vi "PathPlanner_Path_FromJSON.vi"(11 "JSON String":string) -> (0 "Error":bool, 2 "version":string, 3 "PathPlannerPath":T1={"Reversed"=FALSE, "RotationTargets"=[], "ConstraintZones"=[], "EventMarkers"=[], "GlobalConstraints"={"MaxVelocityMps;"=0.0, "MaxAccelerationMpsSq;"=0.0, "MaxAngularVelRadPsEc;"=0.0, "MaxAngularAccRadPSecSq"=0.0, "Exists"=FALSE, "Unlimited"=FALSE, "NominalVoltageVolts"=12.0}, "GoalEndState"={"VelocityMPS"=0.0, "Rotation"={"VALUE"=0.0, "COS"=1.0, "SIN"=0.0}}, "AllPoints"=[], "Name"="", "Waypoints"=[], "PointTowardsZones"=[], "IdealStartingState"={"VelocityMPS"=0.0, "Rotation"={"VALUE"=1.0, "COS"=0.0, "SIN"=0.0}}, "IsChoreoPath"=FALSE, "PreventFlipping"=FALSE} {"IdealStartingState"."Rotation"."SIN" format="%13.4f"; "IdealStartingState"."Rotation"."COS" format="%13.4f"; "IdealStartingState"."Rotation"."VALUE" format="%13.4f"; "PointTowardsZones"."TargetPosition"."Y" format="%14.3f"; "PointTowardsZones"."TargetPosition"."X" format="%14.3f"; "PointTowardsZones"."RotationOffset"."SIN" format="%13.4f"; "PointTowardsZones"."RotationOffset"."COS" format="%13.4f"; "PointTowardsZones"."RotationOffset"."VALUE" format="%13.4f"; "Waypoints"."nextControl"."Y" format="%14.3f"; "Waypoints"."nextControl"."X" format="%14.3f"; "Waypoints"."anchor"."Y" format="%14.3f"; "Waypoints"."anchor"."X" format="%14.3f"; "Waypoints"."prevControl"."Y" format="%14.3f"; "Waypoints"."prevControl"."X" format="%14.3f"; "AllPoints"."RotationTarget"."rotation"."SIN" format="%13.4f"; "AllPoints"."RotationTarget"."rotation"."COS" format="%13.4f"; "AllPoints"."RotationTarget"."rotation"."VALUE" format="%13.4f"; "AllPoints"."Position"."Y" format="%14.3f"; "AllPoints"."Position"."X" format="%14.3f"; "GoalEndState"."Rotation"."SIN" format="%13.4f"; "GoalEndState"."Rotation"."COS" format="%13.4f"; "GoalEndState"."Rotation"."VALUE" format="%13.4f"; "RotationTargets"."rotation"."SIN" format="%13.4f"; "RotationTargets"."rotation"."COS" format="%13.4f"; "RotationTargets"."rotation"."VALUE" format="%13.4f"})   [LabVIEW 2019, in "PathPlanner24.lvlib"]
doc: "Load a path from a JSON string.\n\nInputs: \n - JSON String - string- The string containing the path definition.\n\nOutputs:\n - Path - cluster - PathPlannerPath created from the given JSON string\n - version - string - version string from JSON\n - Error out - cluster - Error cluster\n\n\nNotes:\n--------\nCurrently the only type of commands that can be issued are Boolean commands. The value is forced to TRUE when the command is issued.\n\nThe following table lists the actions performed for different types of commands:\n - Unknown - nothing - not supported.\n - Wait - nothing - not supported\n - Named - Issue boolean command with TRUE value using the \"name\" as the command name.\n - Path - nothing - not supported\n - Sequential, Parallel, Race, Deadline - Issue boolean command with TRUE value for each of the commands contained in the \"commands\" array. The value for \"name\" is used as the command name."
uses:
  PathPlanner24.lvlib
  TypeDef/PathPlannerPath.ctl
  TypeDef/PathPlannerRotationTarget.ctl
  <vilib>/Rock Robotics/WPI/ThirdParty/JAS_Junk/TrajLib/TypeDef/ROTATION2D.ctl
  TypeDef/PathPlannerConstraintsZone.ctl
  TypeDef/PathPlannerPathConstraints.ctl
  TypeDef/PathPlannerEventMarker.ctl
  TypeDef/PathPlannerCommandUtil.ctl
  ENum/PathPlanner_CommandUtil_Type_ENUM.ctl
  TypeDef/PathPlannerGoalEndState.ctl
  TypeDef/PathPlannerPathPoint.ctl
  <vilib>/Rock Robotics/WPI/ThirdParty/JAS_Junk/TrajLib/TypeDef/TRANSLATION2D.ctl
  TypeDef/PathPlannerWaypoint.ctl
  TypeDef/PathPlannerPointTowardsZone.ctl
  TypeDef/PathPlannerIdealStartingState.ctl
  PathPlanner_PointTowardsZone_New.vi
  <vilib>/Rock Robotics/WPI/ThirdParty/JAS_Junk/TrajLib/Rotation2d_CreateAngleDegrees.vi
  <vilib>/Rock Robotics/WPI/ThirdParty/JAS_Junk/TrajLib/Translation2d_Create.vi
  PathPlanner_IdealStartingState_New.vi
  PathPlanner_Waypoint_New.vi
  PathPlanner_GoalEndState_New.vi
  PathPlanner_PathConstraints_New.vi
  <vilib>/Rock Robotics/WPI/ThirdParty/JAS_Junk/TrajLib/Conv_Deg_Radians.vi
  PathPlanner_EventMarker_New.vi
  PathPlanner_CommandUtil_TypeFromString.vi
  PathPlanner_ConstraintsZone_New.vi
  PathPlanner_RotationTarget_New.vi
  <vilib>/Rock Robotics/WPI/ThirdParty/JAS_Junk/TrajLib/Rotation2d_CreateAngle.vi
  PathPlanner_EventMarker_FromJSON_Data.vi
  <vilib>/Rock Robotics/WPI/ThirdParty/JAS_Junk/TrajLib/Trajectory_Library.lvlib
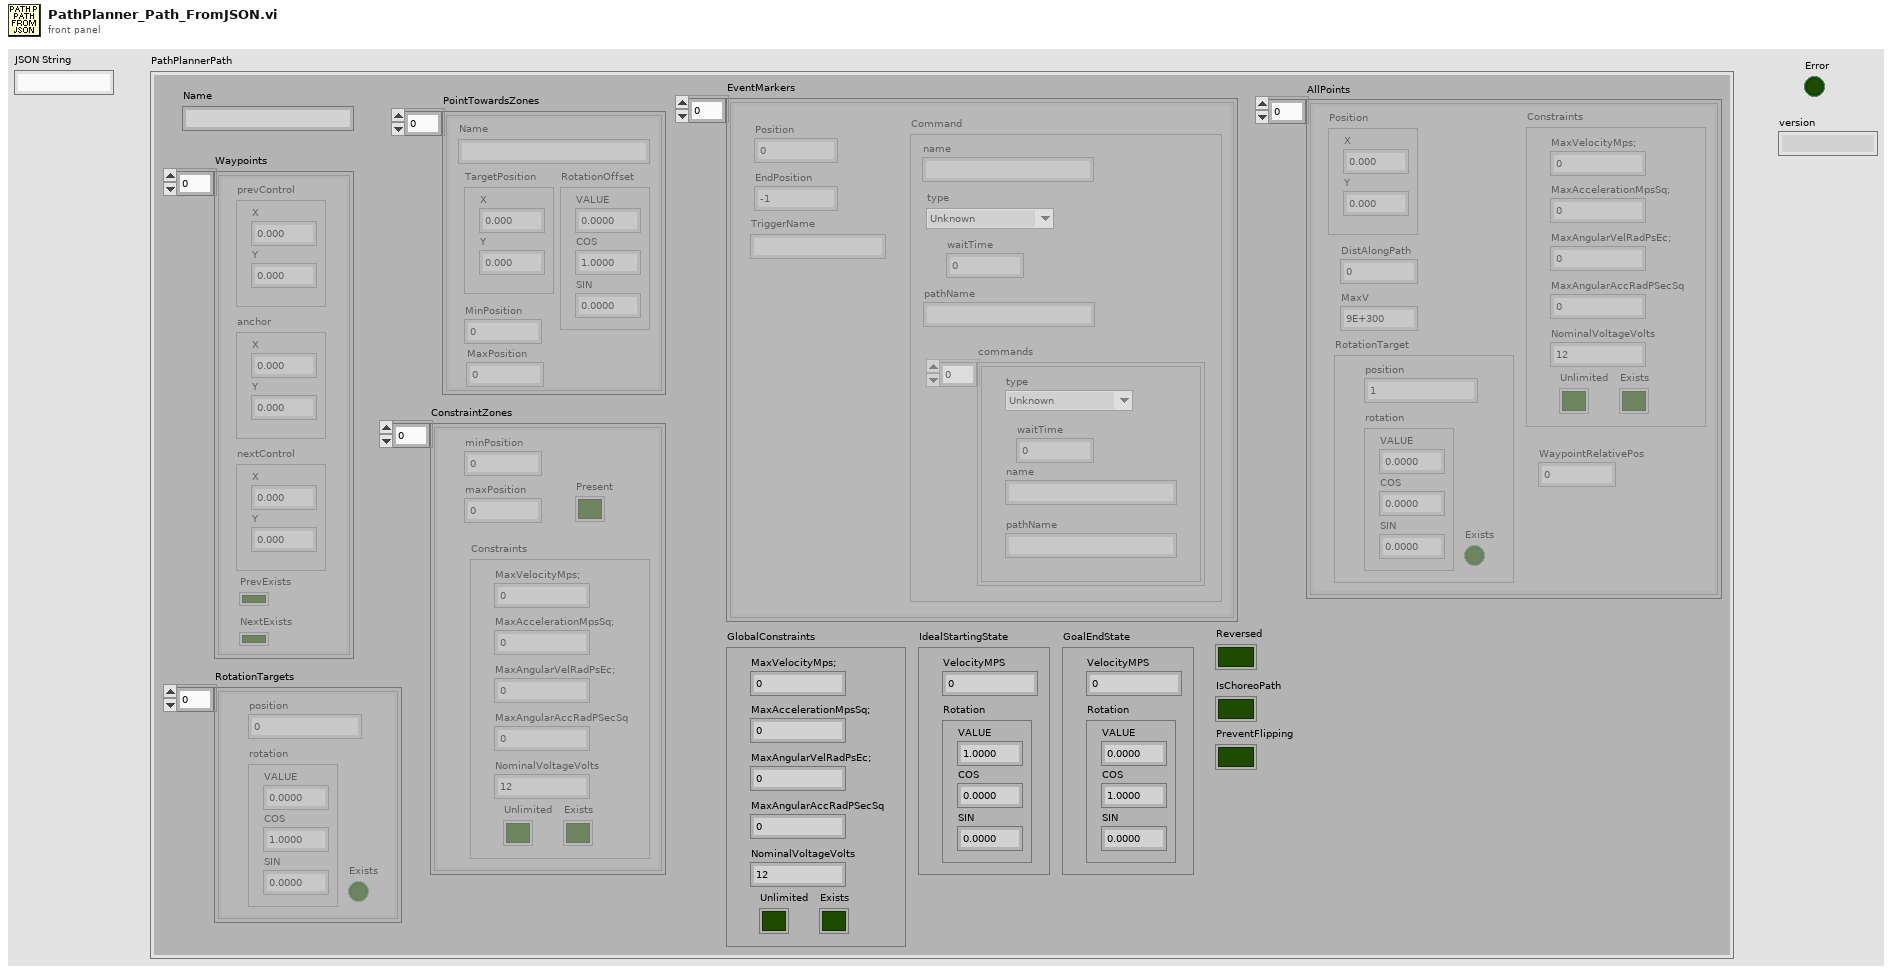
[diagram p1: front panel]
types:
  T1 = typedef "PathPlanner24.lvlib/PathPlannerPath.ctl" = cluster{"Reversed":bool, "RotationTargets":T2[], "ConstraintZones":T4[], "EventMarkers":T6[], "GlobalConstraints":T5, "GoalEndState":T9, "AllPoints":T10[], "Name":string, "Waypoints":T12[], "PointTowardsZones":T13[], "IdealStartingState":T14, "IsChoreoPath":bool, "PreventFlipping":bool}
  T2 = typedef "PathPlanner24.lvlib/PathPlannerRotationTarget.ctl" = cluster{"position":dbl, "rotation":T3, "Exists":bool}
  T3 = typedef "Trajectory_Library.lvlib/ROTATION2D.ctl" = cluster{"VALUE":dbl, "COS":dbl, "SIN":dbl}
  T4 = typedef "PathPlanner24.lvlib/PathPlannerConstraintsZone.ctl" = cluster{"minPosition":dbl, "maxPosition":dbl, "Constraints":T5, "Present":bool}
  T5 = typedef "PathPlanner24.lvlib/PathPlannerPathConstraints.ctl" = cluster{"MaxVelocityMps;":dbl, "MaxAccelerationMpsSq;":dbl, "MaxAngularVelRadPsEc;":dbl, "MaxAngularAccRadPSecSq":dbl, "Exists":bool, "Unlimited":bool, "NominalVoltageVolts":dbl}
  T6 = typedef "PathPlanner24.lvlib/PathPlannerEventMarker.ctl" = cluster{"Position":dbl, "Command":T7, "TriggerName":string, "EndPosition":dbl}
  T7 = typedef "PathPlanner24.lvlib/PathPlannerCommandUtil.ctl" = cluster{"waitTime":dbl, "name":string, "pathName":string, "commands":cluster{"type":T8, "waitTime":dbl, "name":string, "pathName":string}[], "type":T8}
  T8 = typedef "PathPlanner24.lvlib/PathPlanner_CommandUtil_Type_ENUM.ctl" = enum16{"Unknown", "Wait", "Named", "Path", "Sequential", "Parallel", "Race", "Deadline", "PointTowardsZoneEnter", "PointTowardsZoneExit", "TriggerEventStart", "TriggerEventStop", "TriggerEventOneshot"}
  T9 = typedef "PathPlanner24.lvlib/PathPlannerGoalEndState.ctl" = cluster{"VelocityMPS":dbl, "Rotation":T3}
  T10 = typedef "PathPlanner24.lvlib/PathPlannerPathPoint.ctl" = cluster{"Position":T11, "DistAlongPath":dbl, "MaxV":dbl, "Constraints":T5, "RotationTarget":T2, "WaypointRelativePos":dbl}
  T11 = typedef "Trajectory_Library.lvlib/TRANSLATION2D.ctl" = cluster{"X":dbl, "Y":dbl}
  T12 = typedef "PathPlanner24.lvlib/PathPlannerWaypoint.ctl" = cluster{"prevControl":T11, "anchor":T11, "nextControl":T11, "PrevExists":bool, "NextExists":bool}
  T13 = typedef "PathPlanner24.lvlib/PathPlannerPointTowardsZone.ctl" = cluster{"RotationOffset":T3, "Name":string, "TargetPosition":T11, "MinPosition":dbl, "MaxPosition":dbl}
  T14 = typedef "PathPlanner24.lvlib/PathPlannerIdealStartingState.ctl" = cluster{"VelocityMPS":dbl, "Rotation":T3}
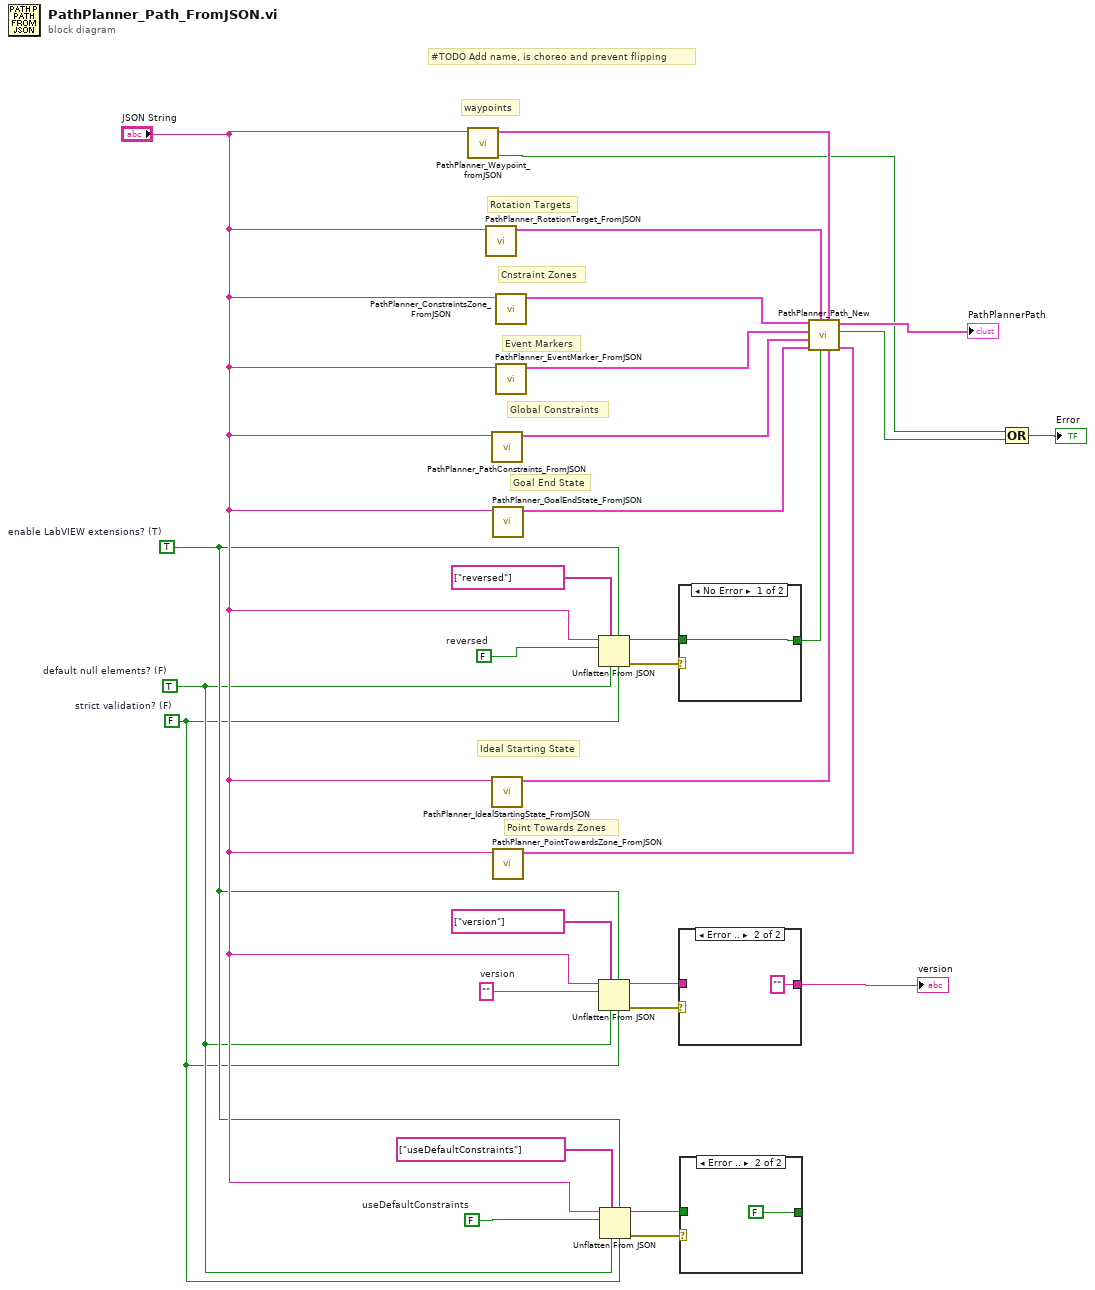
[diagram p0: block diagram]
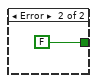
[diagram p4: hidden frame]
diagram:
  w5 = FALSE  # useDefaultConstraints
  w10 = ""  # version
  w2 = FALSE  # strict validation? (F)
  w3 = TRUE  # default null elements? (F)
  w4 = TRUE  # enable LabVIEW extensions? (T)
  w23 = FALSE  # reversed
  # "#TODO Add name, is choreo and prevent flipping"
  # "Point Towards Zones"
  # "Ideal Starting State"
  # "waypoints"
  # "Goal End State"
  # "Global Constraints"
  # "Event Markers"
  # "Cnstraint Zones"
  # "Rotation Targets"
  n1 = call "PathPlanner_Waypoint_fromJSON.vi"("JSON string"="JSON String") -> ("Error"=w17:bool, "waypoints"=w18:T12[])  [unwired: 8 in, 1 out]
  n2 = call "PathPlanner_RotationTarget_FromJSON.vi"("JSON String"="JSON String") -> ("RotationTargets"=w30:T2[])  [unwired: 9 in, 1 out]
  n3 = call "PathPlanner_PathConstraints_FromJSON.vi"("JSON String"="JSON String") -> ("PathPlannerConstraints"=w27:T5)  [unwired: 9 in, 1 out]
  n4 = call "PathPlanner_IdealStartingState_FromJSON.vi"("JSON String"="JSON String") -> ("IdealStartingState"=w16:T14)  [unwired: 9 in, 1 out]
  n5 = call "PathPlanner_GoalEndState_FromJSON.vi"("JSON String"="JSON String") -> ("GoalEndState"=w26:T9)  [unwired: 9 in, 1 out]
  n6 = call "PathPlanner_PointTowardsZone_FromJSON.vi"("JSON String"="JSON String") -> ("PointTowardsZones"=w14:T13[])  [unwired: 9 in, 1 out]
  n7 = call "PathPlanner_ConstraintsZone_FromJSON.vi"("JSON String"="JSON String") -> ("ConstraintZones"=w29:T4[])  [unwired: 9 in, 1 out]
  n8 = call "PathPlanner_EventMarker_FromJSON.vi"("JSON String"="JSON String") -> ("EventMarkers"=w28:T6[])  [unwired: 9 in, 1 out]
  n9 = Unflatten From JSON(path=string[] ["reversed"] ("path 3"), enable LabVIEW extensions? (T)=w4, JSON string="JSON String", type and defaults=w23, default null elements? (F)=w3, strict validation? (F)=w2) -> (value=w19:bool, error out=w21:errorcluster)  [unwired: 1 in]
  n10 = Unflatten From JSON(path=string[] ["version"] ("path 3"), enable LabVIEW extensions? (T)=w4, JSON string="JSON String", type and defaults=w10, default null elements? (F)=w3, strict validation? (F)=w2) -> (value=w11:string, error out=w12:errorcluster)  [unwired: 1 in]
  n11 = Unflatten From JSON(path=string[] ["useDefaultConstraints"] ("path 3"), enable LabVIEW extensions? (T)=w4, JSON string="JSON String", type and defaults=w5, default null elements? (F)=w3, strict validation? (F)=w2) -> (value=w7:bool, error out=w8:errorcluster)  [unwired: 1 in]
  n12 = case shown="No Error" w21 {
    tunnel: [w31 FALSE] -> w20
    tunnel: w19 -> [w31 _]
    frame No Error {
    }
    frame Error {
    }
  }
  n13 = case shown="Error .." w12 {
    tunnel: [w33 "" ("version")] -> w1
    tunnel: w11 -> [w33 _]
    frame No Error {
    }
    frame Error {
    }
  }
  "version" <- w1
  n14 = case shown="Error .." w8 {
    tunnel: [w35 FALSE] -> _
    tunnel: w7 -> [w35 _]
    frame No Error {
    }
    frame Error {
    }
  }
  n15 = call "PathPlanner_Path_New.vi"("PointTowardsZones"=w14, "IdealStartingState"=w16, "Waypoints"=w18, "Reversed"=w20, "HolonomicRotations"=w30, "GoalEndState"=w26, "GlobalConstraints"=w27, "EventMarkers"=w28, "ConstraintZones"=w29) -> ("Error"=w15:bool, "PathPlannerPath"=→"PathPlannerPath":T1)  [unwired: 1 in]
  n16 = Compound Arithmetic op=OR(w17, w15) -> (→"Error":bool)
